vi "TDMSWrite(SubVI)_7ch.vi"(0 "tdms file out 입력":refnum<k34>, 1 "배열":dbl[](array[numeric]), 5 "그룹입력":string="Robot-M1509", 7 "채널입력":string[](array[string]), 11 "에러 입력":errorcluster caption="에러 입력(에러 없음)") -> (4 "참조 번호 출력":refnum<k34>, 15 "에러 출력":errorcluster)   [LabVIEW 2019]
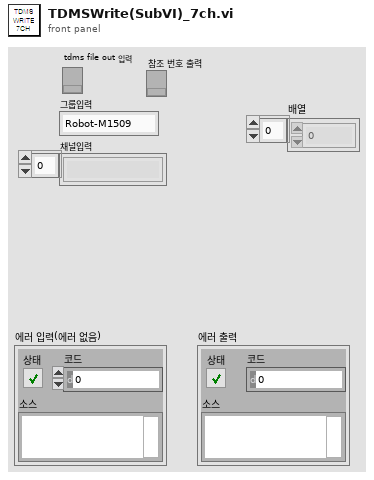
[diagram p1: front panel]
types:
  T1 = cluster{"배열[0]":dbl, "배열[1]":dbl, "배열[2]":dbl, "배열[3]":dbl, "배열[4]":dbl, "배열[5]":dbl, "배열[6]":dbl, "배열[7]":dbl, "배열[8]":dbl}
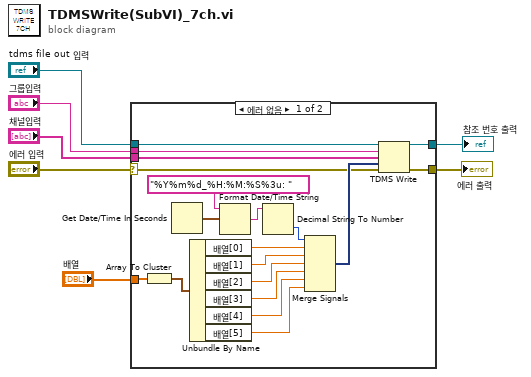
[diagram p0: block diagram]
diagram:
  n1 = case shown="에러 없음" "에러 입력" {
    selector: "에러 입력" -> [w22 w27]
    tunnel: [w25 w28] -> w7
    tunnel: [w24 w27] -> w6
    tunnel: "tdms file out 입력" -> [w23 w28]
    tunnel: "그룹입력" -> [w21 _]
    tunnel: "채널입력" -> [w20 _]
    tunnel: "배열" -> [w19 _]
    frame No Error {
      n2 = Array To Cluster(array=w19) -> (cluster=w18:T1)
      n3 = Get Date/Time In Seconds() -> (seconds since 1Jan1904=w11:timestamp)
      n4 = Unbundle By Name(w18) -> ("배열[0]"=w17:dbl, "배열[1]"=w16:dbl, "배열[2]"=w15:dbl, "배열[3]"=w14:dbl, "배열[4]"=w10:dbl, "배열[5]"=w9:dbl)
      n5 = Format Date/Time String(time format string (%c)="%Y%m%d_%H:%M:%S%3u: " ("시간 포맷 문자열 (%c)"), seconds (now)=w11) -> (date/time string=w13:string)  [unwired: 1 in]
      n6 = Decimal String To Number(string=w13) -> (number=w12:i32)  [unwired: 2 in, 1 out]
      n7 = Merge Signals(w12, w17, w16, w15, w14, w10, w9) -> (w26:dynamicdata)
      n8 = TDMS Write(0:w23, 5:w21, 7:w20, 9:w26, 11:w22) -> (4:w25:refnum<k34>, 15:w24:errorcluster)  [unwired: 1 in, 2 out]
    }
    frame Error {
    }
  }
  "참조 번호 출력" <- w7
  "에러 출력" <- w6
